vi "Show Binary.vi"(0 "Input Image":T1(plugin-control), 5 "LUT1":cluster{u16, u16}(slide)={0, 4095} caption="Slide" scale=0.0..4095.0, 7 "Boundary":dbl, 11 "error in (no error)":errorcluster) -> (4 "Binary Image":T1(plugin-control), 6 "Reference Rectangles":i16[][](array[numeric]), 8 "Reference CoM":i16[][](array[numeric]), 10 "Histogram Graph":T2 {"Incremental Value" format="%.2f"; "Starting Value" format="%.2f"}, 14 "Number of Particles":i32, 15 "error out":errorcluster)   [LabVIEW 2020]
uses:
  <vilib>/vision/Image Controls.llb/IMAQ Image.ctl
  <vilib>/vision/NI_Vision_Development_Module.lvlib
panel:
  out "got copy":bool=TRUE
  out "upper":u16
  out "lower":u16
  out "Mean Value":sgl format="%.2f"
  out "temp copy":T1
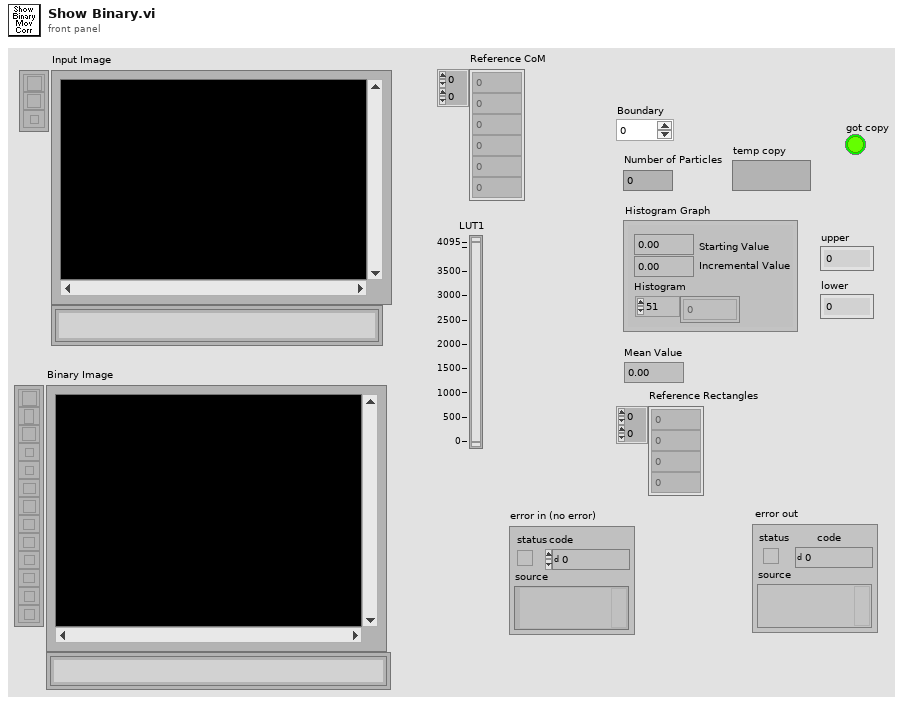
[diagram p1: front panel]
types:
  T1 = typedef "IMAQ Image.ctl" = refnum<image>
  T2 = cluster{"Starting Value":sgl, "Incremental Value":sgl, "Histogram":u32[]}
  T3 = cluster{"Left":i32, "Top":i32, "Right":i32, "Bottom":i32}
  T4 = typedef "Particle Parameters" = i32
  T5 = typedef "Image Type" = u32
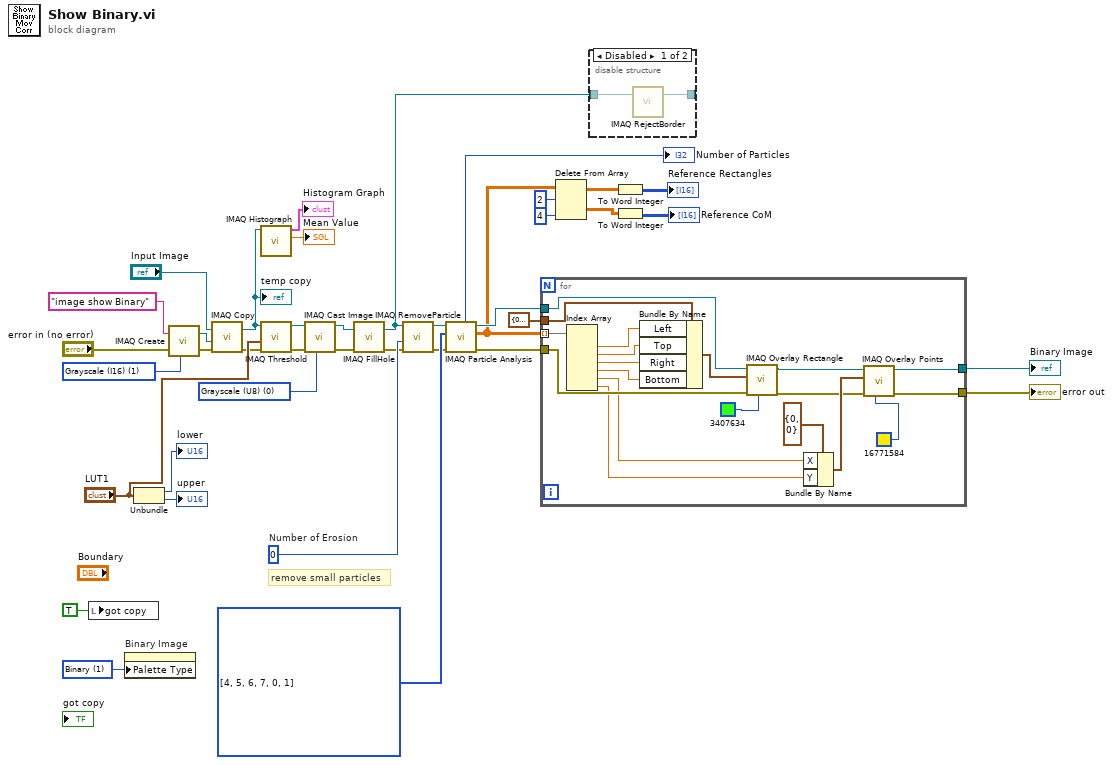
[diagram p0: block diagram]
diagram:
  w22 = u32 1 items=["Grayscale", "Binary", "Gradient", "Rainbow", "Temperature", "User Defined"] ("Palette:Palette Type")
  w28 = T4[] [4, 5, 6, 7, 0, 1] items=["Center of Mass X", "Center of Mass Y", "First Pixel X", "First Pixel Y", "Bounding Rect Left", "Bounding Rect Top", "Bounding Rect Right", "Bounding Rect Bottom", "Max Feret Diameter Start X", "Max Feret Diameter Start Y", "Max Feret Diameter End X", "Max Feret Diameter End Y", "Max Horiz. Segment Length Left", "Max Horiz. Segment Length Right", "Max Horiz. Segment Length Row", "-", "Bounding Rect Width", "Bounding Rect Height", "Bounding Rect Diagonal", "Perimeter", "Convex Hull Perimeter", "Holes' Perimeter", "Max Feret Diameter", "Equivalent Ellipse Major Axis", "Equivalent Ellipse Minor Axis", "Equivalent Ellipse Minor Axis (Feret)", "Equivalent Rect Long Side", "Equivalent Rect Short Side", "Equivalent Rect Diagonal", "Equivalent Rect Short Side (Feret)", "Average Horiz. Segment Length", "Average Vert. Segment Length", "Hydraulic Radius", "Waddel Disk Diameter", "-", "Area", "Holes' Area", "Particle & Holes' Area", "Convex Hull Area", "Image Area", "-", "Number of Holes", "Number of Horiz. Segments", "Number of Vert. Segments", "-", "Orientation", "Max Feret Diameter Orientation", "-", "% Area/Image Area", "% Area/(Particle & Holes' Area)", "Ratio of Equivalent Ellipse Axes", "Ratio of Equivalent Rect Sides", "-", "Elongation Factor", "Compactness Factor", "Heywood Circularity Factor", "Type Factor", "-", "Sum X", "Sum Y", "Sum XX", "Sum XY", "Sum YY", "Sum XXX", "Sum XXY", "Sum XYY", "Sum YYY", "-", "Moment of Inertia XX", "Moment of Inertia XY", "Moment of Inertia YY", "Moment of Inertia XXX", "Moment of Inertia XXY", "Moment of Inertia XYY", "Moment of Inertia YYY", "Norm. Moment of Inertia XX", "Norm. Moment of Inertia XY", "Norm. Moment of Inertia YY", "Norm. Moment of Inertia XXX", "Norm. Moment of Inertia XXY", "Norm. Moment of Inertia XYY", "Norm. Moment of Inertia YYY", "Hu Moment 1", "Hu Moment 2", "Hu Moment 3", "Hu Moment 4", "Hu Moment 5", "Hu Moment 6", "Hu Moment 7"] ("Pixel Measurements")
  w29 = 0  # Number of Erosion
  w30 = T5 0 items=["Grayscale (U8)", "Grayscale (I16)", "Grayscale (SGL)", "Complex (CSG)", "RGB (U32)", "HSL (U32)", "RGB (U64)", "Grayscale (U16)"] ("Image Type")
  w38 = T5 1 items=["Grayscale (U8)", "Grayscale (I16)", "Grayscale (SGL)", "Complex (CSG)", "RGB (U32)", "HSL (U32)", "RGB (U64)", "Grayscale (U16)"] ("Image Type")
  # "remove small particles"
  n1 = local write "got copy"(TRUE) -> ()
  n2 = property on="Binary Image" class="ImageControl"("Palette Type"=w22) -> ()  [unwired: 2 in, 2 out]
  n3 = Unbundle("LUT1") -> (→"lower":u16, →"upper":u16)
  n4 = call "IMAQ Create"("Image Name"="image show Binary", "Image Type"=w38, "error in (no error)"="error in (no error)") -> ("New Image"=w37:T1, "error out"=w9:errorcluster)  [unwired: 2 in]
  n5 = call "IMAQ Copy"("error in (no error)"=w9, "Image Dst"=w37, "Image Src"="Input Image") -> ("error out"=w10:errorcluster, "Image Dst Out"=w33:T1)  [unwired: 3 in]
  "temp copy" <- w33
  n6 = call "IMAQ Histograph"("Image"=w33) -> ("Mean Value"=→"Mean Value":sgl, "Histogram Graph"=→"Histogram Graph":T2)  [unwired: 7 in, 2 out]
  n7 = call "IMAQ Threshold"("error in (no error)"=w10, "Range"="LUT1", "Image Src"=w33) -> ("error out"=w11:errorcluster, "Image Dst Out"=w32:T1)  [unwired: 3 in, 4 out]
  n8 = call "IMAQ Cast Image"("Image Type"=w30, "error in (no error)"=w11, "Image Src"=w32) -> ("error out"=w12:errorcluster, "Image Dst Out"=w31:T1)  [unwired: 7 in]
  n9 = call "IMAQ FillHole"("error in (no error)"=w12, "Image Src"=w31) -> ("error out"=w13:errorcluster, "Image Dst Out"=w21:T1)  [unwired: 2 in, 2 out]
  n10 = call "IMAQ RemoveParticle"("error in (no error)"=w13, "Number of Erosion"=w29, "Image Src"=w21) -> ("error out"=w14:errorcluster, "Image Dst Out"=w20:T1)  [unwired: 4 in, 3 out]
  n11 = call "IMAQ Particle Analysis"("error in (no error)"=w14, "Pixel Measurements"=w28, "Image"=w20) -> ("error out"=w15:errorcluster, "Particle Measurements (Pixels)"=w3:dbl[][], "Image Out (duplicate)"=w27:T1, "Number of Particles"=→"Number of Particles":i32)  [unwired: 3 in, 2 out]
  n12 = for {
    tunnel: [w44] -> w18
    tunnel: w27 -> [w57]
    tunnel: w3 -> [w55] mode=indexing
    tunnel: T3 {"Left"=0, "Top"=0, "Right"=0, "Bottom"=0} ("Rectangle") -> [w56]
    tunnel: [w43] -> w16
    tunnel: w15 -> [w49]
    n13 = Index Array(array=w55) -> (element #1=w53:dbl, element #2=w52:dbl, element #3=w51:dbl, element #4=w50:dbl, element #5=w41:dbl, element #6=w40:dbl)  [unwired: 6 in]
    n14 = Bundle By Name(cluster=w56, "Left"=w53, "Top"=w52, "Right"=w51, "Bottom"=w50) -> (w54:T3)
    n15 = call "IMAQ Overlay Rectangle"("Color"=u32 3407634 ("Text Color (black)"), "error in (no error)"=w49, "Rectangle"=w54, "Image"=w57) -> ("error out"=w45:errorcluster, "Image Out"=w46:T1)  [unwired: 6 in]
    n16 = Bundle By Name(cluster=cluster{"X":i32, "Y":i32} {"X"=0, "Y"=0} ("Point"), "X"=w41, "Y"=w40) -> (w48:cluster{"X":i32, "Y":i32})
    n17 = call "IMAQ Overlay Points"("Color"=u32 16771584 ("Text Color (black)"), "error in (no error)"=w45, "Point"=w48, "Image"=w46) -> ("error out"=w43:errorcluster, "Image Out"=w44:T1)  [unwired: 6 in]
  }
  "Binary Image" <- w18
  "error out" <- w16
  n18 = Delete From Array(array=w3, length=2, index (col)=4 ("disabled index (col)")) -> (deleted portion=w4:dbl[][], array with subset deleted=w5:dbl[][])  [unwired: 1 in]
  n19 = disable-structure shown="Disabled" {
    disable-tunnel: w21 -> [w60 _]
    disable-tunnel: [w59 _] -> _
    frame Disabled {
      n20 = call "IMAQ RejectBorder"("Image Src"=w60) -> ("Image Dst Out"=w59:T1)  [unwired: 3 in, 3 out]
    }
    frame Enabled {
    }
  }
  n21 = To Word Integer(number=w5) -> (16bit integer=→"Reference Rectangles":i16[][])
  n22 = To Word Integer(number=w4) -> (16bit integer=→"Reference CoM":i16[][])
